vi "Initialize.vi"(0 "TCP Socket In":refnum<class "Socket Communication.lvclass">, 5 "error in (no error)":errorcluster) -> (14 "TCP Socket Out":refnum<class "Socket Communication.lvclass">, 19 "error out":errorcluster)   [LabVIEW 2019, in "Socket Communication.lvclass"]
uses:
  Socket Communication.lvclass
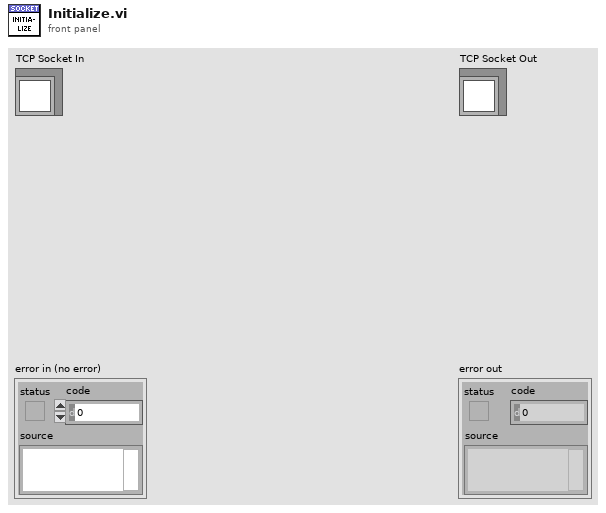
[diagram p1: front panel]
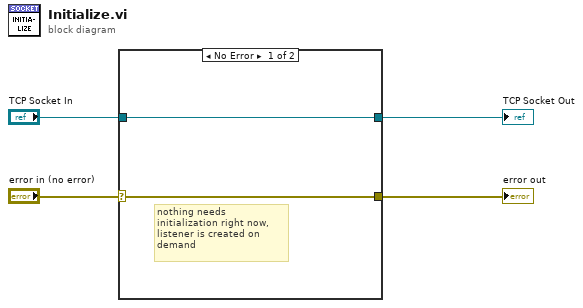
[diagram p0: block diagram]
diagram:
  n1 = case shown="No Error" "error in (no error)" {
    selector: "error in (no error)" -> [w6 w8]
    tunnel: [w6 w8] -> w4
    tunnel: [w5 w7] -> w3
    tunnel: "TCP Socket In" -> [w5 w7]
    frame No Error {
      # "nothing needs initialization right now, listener is created on demand"
    }
    frame Error {
    }
  }
  "error out" <- w4
  "TCP Socket Out" <- w3
